vi "Dequeue_Message.vi"(8 "error in (no error)":errorcluster={"status"=FALSE, "code"=0, "source"="\"\""}, 11 "Message Queue":refnum<queue>) -> (0 "error out":errorcluster, 2 "Message":string, 3 "dup Message Queue":refnum<queue>)   [LabVIEW 2026]
doc: "Pulls message from queue, traps errors and returns Exit message on error to stop loop cleanly."
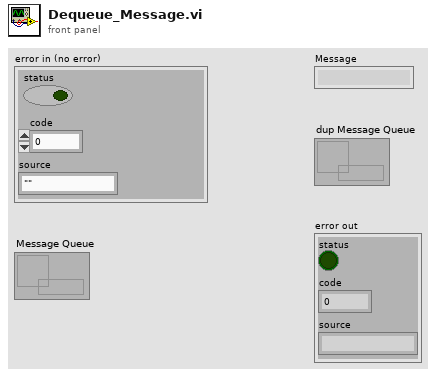
[diagram p1: front panel]
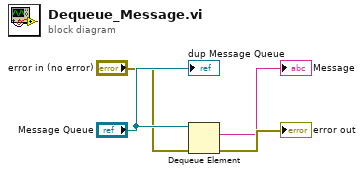
[diagram p0: block diagram]
diagram:
  n1 = Dequeue Element(queue="Message Queue", error in (no error)="error in (no error)") -> (element=→"Message":string, error out=→"error out":errorcluster)  [unwired: 1 in, 2 out]
  "dup Message Queue" <- "Message Queue"
